vi "Insert Into Replacement Map.vi"(9 "Replace Value":u16, 10 "Replace Column":T1, 11 "Replace Map":map{T1, u16}(c390)) -> (3 "Replace Map out":map{T1, u16}(c390))   [LabVIEW 2020, in "VI Properties Editor.lvlib"]
doc: "Inserts into <B>Replace Map</B> the key-value pair of <B>Replace Column</B> and <B>Replace Value</B>."
uses:
  VI Properties Editor.lvlib
  CTLs/Replace Column.ctl
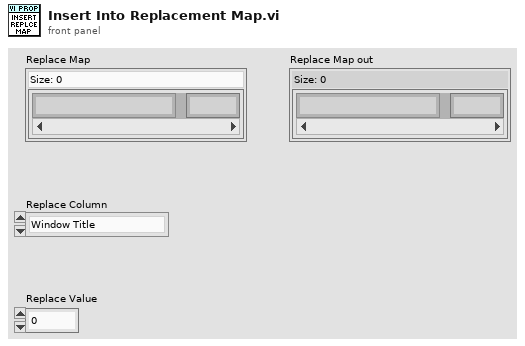
[diagram p1: front panel]
types:
  T1 = typedef "VI Properties Editor.lvlib/Replace Column.ctl" = enum16{"Window Title", "Description", "Help Path", "Help Tag", "Custom Title?", "Help URL", "Help Type", "Inlined?", "Allow debugging?", "Auto error handling?", "Run when opened?", "Suspend when called?", "Reentrancy", "Priority", "Preferred Exec System", "Control Label", "Control Caption", "Control Description", "Control Tip Strip"}
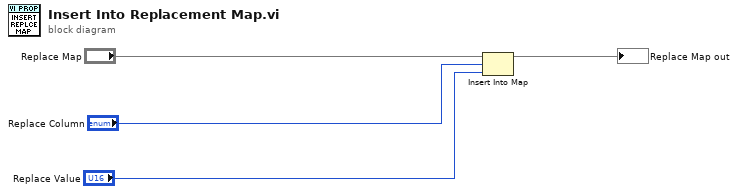
[diagram p0: block diagram]
diagram:
  n1 = Insert Into Map(map in="Replace Map", key="Replace Column", value="Replace Value") -> (map out=→"Replace Map out":map{T1, u16})  [unwired: 2 out]
